vi "SQL_Connect_MSOLEDBSQL.vi"(4 "Passwort":string, 6 "User Name":string, 8 "error in (no error)":errorcluster caption="Fehler (Eingang, kein Fehler)", 10 "Database Name":string, 11 "Server Name":string) -> (0 "error out":errorcluster caption="Fehler (Ausgang)", 3 "Connection String":string)   [LabVIEW 2024, in "DB-Tool.lvlib"]
doc: "Erzeugt einen Connection String mit dem Treiber MSOLEDBSQL, ist der Treiber nicht installiert wird ein leerer Connection string ausgegeben."
uses:
  DB-Tool.lvlib
panel:
  # "Connector Pane"
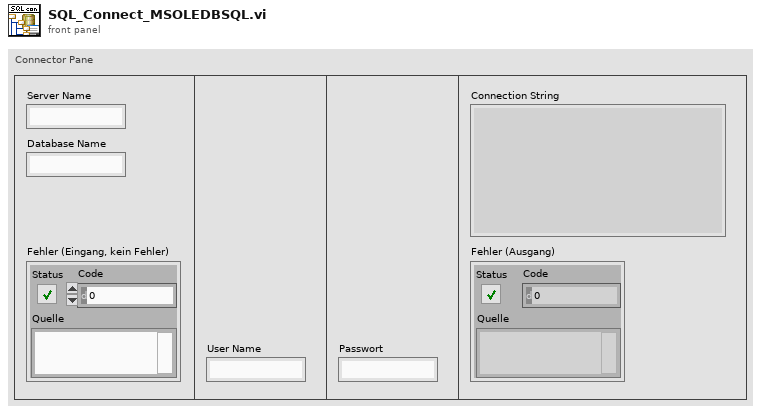
[diagram p1: front panel]
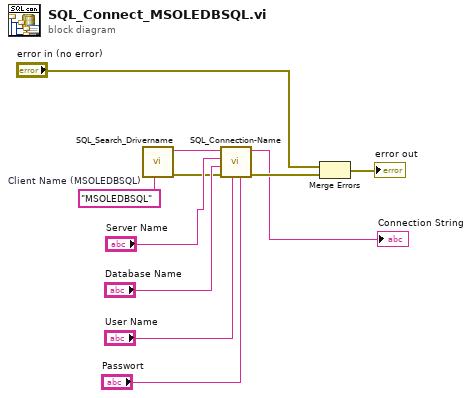
[diagram p0: block diagram]
diagram:
  w1 = "MSOLEDBSQL"  # Client Name (MSOLEDBSQL)
  n1 = call "SQL_Search_Drivername.vi"("Client Name (MSOLEDBSQL)"=w1) -> ("error out"=w6:errorcluster, "Client Name"=w11:string)  [unwired: 7 in, 2 out]
  n2 = call "SQL_Connection-Name.vi"("Passwort"="Passwort", "User Name"="User Name", "error in (no error)"=w6, "Database Name"="Database Name", "Server Name"="Server Name", "SQL Driver  Clientname"=w11) -> ("error out"=w5:errorcluster, "Connection String"=→"Connection String":string)  [unwired: 4 in]
  n3 = Merge Errors("error in (no error)", w5) -> (→"error out":errorcluster)
